vi "Render Set Clip Rect.vi"(8 "error in":errorcluster, 10 "Rectangle":T1, 11 "Renderer Pointer":u32 format="%.0x") -> (0 "error out":errorcluster, 3 "Return":i32)   [LabVIEW 2021, in "LibSDL2.lvlib"]
uses:
  LibSDL2.lvlib
  DLL/SDL2.dll
  Controls/Rectangle.ctl
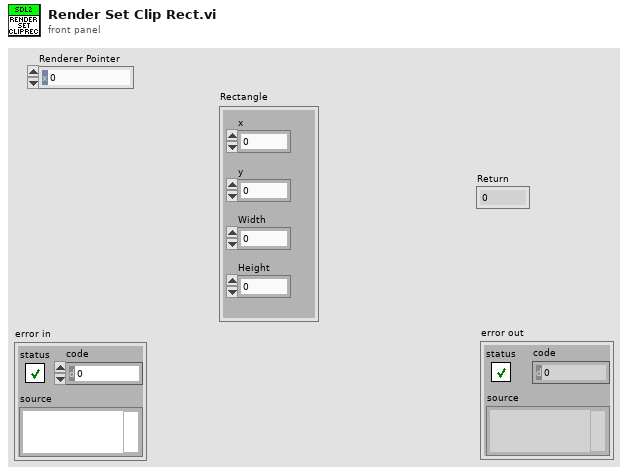
[diagram p1: front panel]
types:
  T1 = typedef "LibSDL2.lvlib/Rectangle.ctl" = cluster{"x":i32, "y":i32, "Width":i32, "Height":i32}
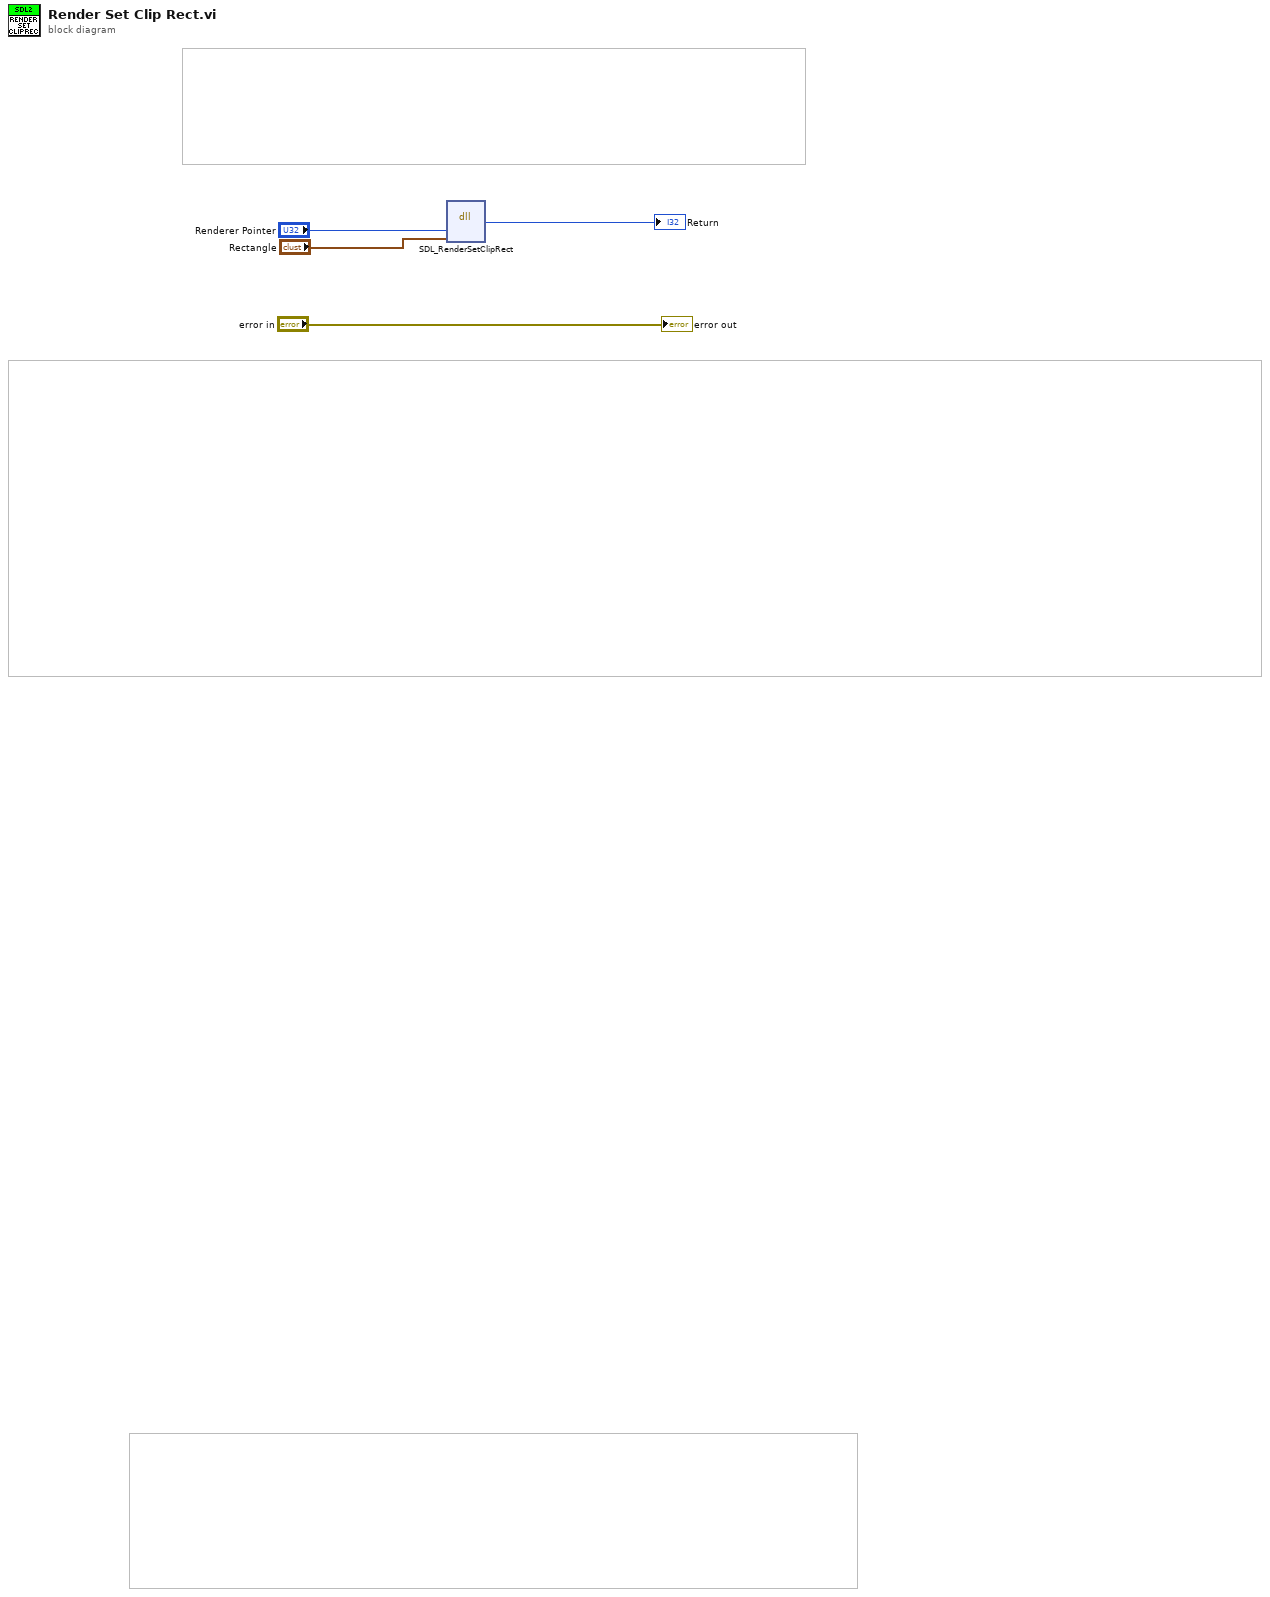
[diagram p0: block diagram]
diagram:
  n1 = dll-call lib="C:/dev/LabVIEW/LabSDL2/Source/Libraries/LibSDL2 Wrapper/DLL/SDL2.dll" fn="SDL_RenderSetClipRect"("renderer_pointer"="Renderer Pointer", "rect_pointer"="Rectangle") -> ("return type"=→"Return":i32)  [unwired: 5 in, 2 out]
  "error out" <- "error in"
